vi "test Get All Parameters.vi"(8 "error in":errorcluster, 11 "TestCase in":refnum<class "Scripting.lvclass">) -> (0 "error out":errorcluster, 3 "TestCase out":refnum<class "Scripting.lvclass">)   [LabVIEW 2020, in "Scripting.lvclass"]
uses:
  Scripting.lvclass
  <vilib>/addons/_JKI Toolkits/VI Tester/TestCase.llb/TestCase.lvclass
  Scripting/AIM/AIM ARINC 429 Scripting.lvlib
  Shared/Transfer Type.ctl
  <vilib>/NI/NI VeriStand Encoding and Decoding/Encoding.ctl
  <vilib>/NI/NI VeriStand Encoding and Decoding/Encoding and Decoding.lvlib
  Shared/Parameter Definition.ctl
  Shared/VS Channel Definition for Parameter.ctl
  Shared/VS Channels Definition for Label.ctl
  Shared/Direction.ctl
  Shared/Transfer Speed.ctl
  C:/Program Files (x86)/National Instruments/LabVIEW 2020/vi.lib/addons/_JKI Toolkits/VI Tester/TestCase.llb/TestCase.lvclass
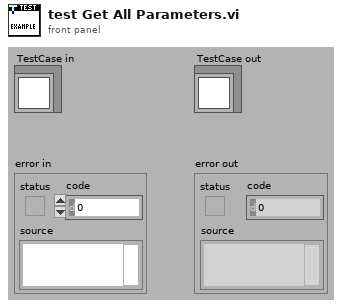
[diagram p1: front panel]
types:
  T1 = typedef "VS Channels Definition for Label.ctl" = cluster{"label (Dec)":u32, "parameters":T2[], "SDI value":u8, "SDI enabled":bool, "transfer type":T5, "create timestamp":bool, "transmit period":u32}
  T2 = typedef "VS Channel Definition for Parameter.ctl" = cluster{"name":string, "unit":string, "Parameter":T3}
  T3 = typedef "Parameter Definition.ctl" = cluster{"start index":i32, "size":i32, "encoding":T4, "signed":bool, "scale multiplier":dbl, "scale offset":dbl, "default value":dbl}
  T4 = typedef "Encoding and Decoding.lvlib/Encoding.ctl" = enum16{"BNR", "BCD", "Discrete"}
  T5 = typedef "Transfer Type.ctl" = enum16{"Scheduled", "Acyclic", "Block", "Strobe"}
  T6 = typedef "Transfer Speed.ctl" = enum16{"LO (12.5 kb/s)", "HI (100 kb/s)"}
  T7 = typedef "Direction.ctl" = enum16{"Rx", "Tx"}
  T8 = typedef "Custom Device API.lvlib/Custom Device Item Ref.ctl" = u64
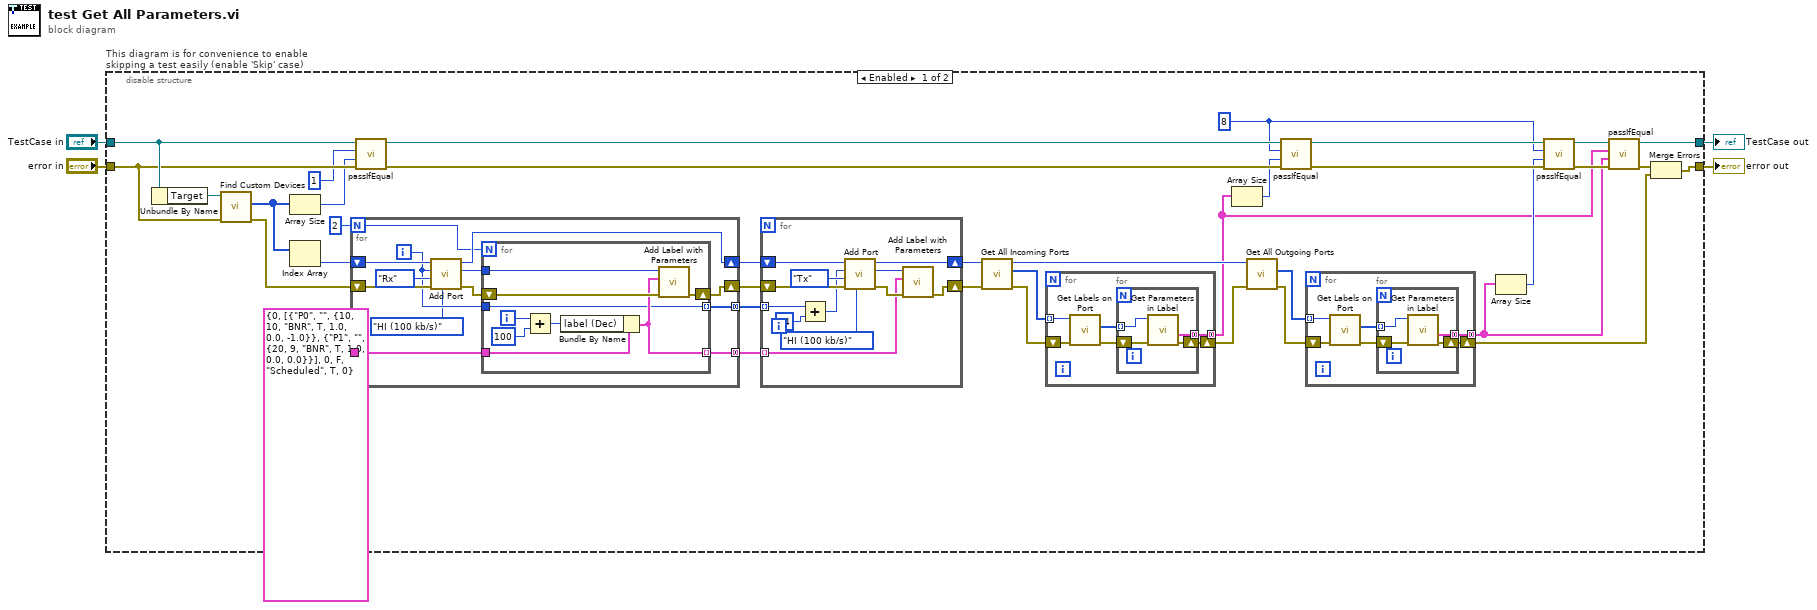
[diagram p0: block diagram]
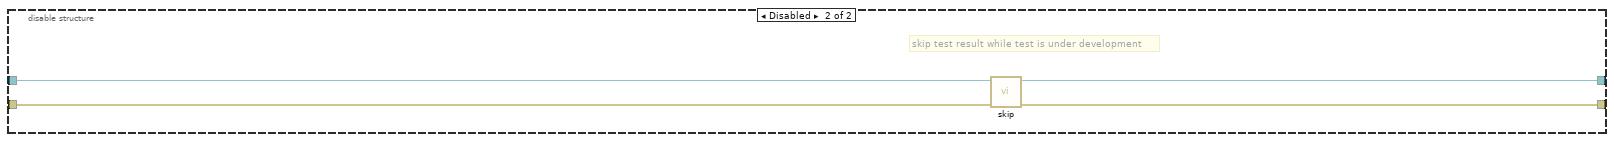
[diagram p2: hidden frame]
diagram:
  n1 = disable-structure "This diagram is for convenience to enable skipping a test easily (enable 'Skip' case)" shown="Enabled" {
    disable-tunnel: "TestCase in" -> [w40 w99]
    disable-tunnel: [w32 w97] -> w1
    disable-tunnel: [w33 w98] -> w3
    disable-tunnel: "error in" -> [w39 w96]
    frame Enabled {
      w7 = 8 ("size(s)")
      n2 = Unbundle By Name(w40) -> ("Target"=w41:refnum<k24>)
      n3 = call "Find Custom Devices.vi"("error in"=w39, "target in"=w41) -> ("error out"=w15:errorcluster, "AIM ARINC 429 custom devices"=w18:u64[])  [unwired: 7 in, 1 out]
      n4 = Array Size(array=w18) -> (size(s)=w37:i32)
      n5 = Index Array(array=w18) -> (element=w17:u64)  [unwired: 1 in]
      n6 = for {
        N: 2 -> [w55]
        shift-right: [w60] -> w11
        shift-left: w17 -> [w64]
        shift-right: [w61] -> w10
        shift-left: w15 -> [w62]
        tunnel: T1 {"label (Dec)"=0, "parameters"=[{"name"="P0", "unit"="", "Parameter"={"start index"=10, "size"=10, "encoding"=enum."BNR", "signed"=TRUE, "scale multiplier"=1.0, "scale offset"=0.0, "default value"=-1.0}}, {"name"="P1", "unit"="", "Parameter"={"start index"=20, "size"=9, "encoding"=enum."BNR", "signed"=TRUE, "scale multiplier"=1.0, "scale offset"=0.0, "default value"=0.0}}], "SDI value"=0, "SDI enabled"=FALSE, "transfer type"=enum."Scheduled", "create timestamp"=TRUE, "transmit period"=0} ("label") -> [w59]
        tunnel: [w58] -> w9 mode=concatenating
        tunnel: [w56] -> w8 mode=concatenating
        i -> [w57]
        n7 = call "Add Port.vi"("speed"=Transfer_Speed."HI (100 kb/s)", "error in"=w62, "direction"=Direction."Rx", "port number"=w57, "AIM ARINC 429 custom device in"=w64) -> ("error out"=w65:errorcluster, "port"=w66:T8, "AIM ARINC 429 custom device out"=w60:T8)  [unwired: 4 in]
        n8 = for {
          N: w55 -> [_]
          tunnel: w66 -> [w75]
          shift-right: [w73] -> w61
          shift-left: w65 -> [w74]
          tunnel: w59 -> [w72]
          tunnel: [w71] -> w58 mode=indexing
          tunnel: w57 -> [w67]
          tunnel: [w67] -> w56 mode=indexing
          i -> [w70]
          n9 = Add(x=w70, y=100) -> (x+y=w69:i32)
          n10 = Bundle By Name(cluster=w72, "label (Dec)"=w69) -> (w71:T1)
          n11 = call "Add Label with Parameters.vi"("error in"=w74, "label"=w71, "port ref"=w75) -> ("error out"=w73:errorcluster)  [unwired: 7 in, 1 out]
        }
      }
      n12 = call-dynamic "passIfEqual.vi"("error in (no error)"=w39, "y"=w37, "x"=1 ("size(s)"), "TestCase in"=w40) -> ("error out"=w35:errorcluster, "TestCase out"=w36:refnum<class "Scripting.lvclass">)  [unwired: 6 in]
      n13 = for {
        shift-right: [w50] -> w13
        shift-left: w11 -> [w51]
        shift-right: [w47] -> w12
        shift-left: w10 -> [w48]
        tunnel: w9 -> [w44] mode=indexing
        tunnel: w8 -> [w43] mode=indexing
        n14 = Add(x=w43, y=24 ("x")) -> (x+y=w45:i32)
        n15 = call "Add Port.vi"("speed"=Transfer_Speed."HI (100 kb/s)", "error in"=w48, "direction"=Direction."Tx", "port number"=w45, "AIM ARINC 429 custom device in"=w51) -> ("error out"=w52:errorcluster, "port"=w53:T8, "AIM ARINC 429 custom device out"=w50:T8)  [unwired: 4 in]
        n16 = call "Add Label with Parameters.vi"("error in"=w52, "label"=w44, "port ref"=w53) -> ("error out"=w47:errorcluster)  [unwired: 7 in, 1 out]
      }
      n17 = call "Get All Incoming Ports.vi"("error in"=w12, "AIM ARINC 429 custom device in"=w13) -> ("error out"=w27:errorcluster, "incoming ports"=w26:T8[], "AIM ARINC 429 custom device out"=w34:T8)  [unwired: 7 in]
      n18 = for {
        tunnel: [w90] -> w5 mode=concatenating
        shift-right: [w91] -> w30
        shift-left: w27 -> [w89]
        tunnel: w26 -> [w86] mode=indexing
        n19 = call "Get Labels on Port.vi"("error in"=w89, "port in"=w86) -> ("error out"=w88:errorcluster, "labels"=w87:T8[])  [unwired: 6 in, 2 out]
        n20 = for {
          tunnel: [w94] -> w90 mode=concatenating
          shift-right: [w95] -> w91
          shift-left: w88 -> [w93]
          tunnel: w87 -> [w92] mode=indexing
          n21 = call "Get Parameters in Label.vi"("error in"=w93, "label in"=w92) -> ("error out"=w95:errorcluster, "parameter definitions"=w94:T3[])  [unwired: 6 in, 2 out]
        }
      }
      n22 = Array Size(array=w5) -> (size(s)=w20:i32)
      n23 = call "Get All Outgoing Ports.vi"("error in"=w30, "AIM ARINC 429 custom device in"=w34) -> ("error out"=w22:errorcluster, "outgoing ports"=w23:T8[])  [unwired: 7 in, 1 out]
      n24 = call-dynamic "passIfEqual.vi"("error in (no error)"=w35, "y"=w20, "x"=w7, "TestCase in"=w36) -> ("error out"=w28:errorcluster, "TestCase out"=w29:refnum<class "Scripting.lvclass">)  [unwired: 6 in]
      n25 = for {
        tunnel: [w80] -> w6 mode=concatenating
        shift-right: [w81] -> w21
        shift-left: w22 -> [w79]
        tunnel: w23 -> [w76] mode=indexing
        n26 = call "Get Labels on Port.vi"("error in"=w79, "port in"=w76) -> ("error out"=w78:errorcluster, "labels"=w77:T8[])  [unwired: 6 in, 2 out]
        n27 = for {
          tunnel: [w84] -> w80 mode=concatenating
          shift-right: [w85] -> w81
          shift-left: w78 -> [w83]
          tunnel: w77 -> [w82] mode=indexing
          n28 = call "Get Parameters in Label.vi"("error in"=w83, "label in"=w82) -> ("error out"=w85:errorcluster, "parameter definitions"=w84:T3[])  [unwired: 6 in, 2 out]
        }
      }
      n29 = Array Size(array=w6) -> (size(s)=w19:i32)
      n30 = call-dynamic "passIfEqual.vi"("error in (no error)"=w28, "y"=w19, "x"=w7, "TestCase in"=w29) -> ("error out"=w24:errorcluster, "TestCase out"=w25:refnum<class "Scripting.lvclass">)  [unwired: 6 in]
      n31 = call-dynamic "passIfEqual.vi"("error in (no error)"=w24, "y"=w6, "x"=w5, "TestCase in"=w25) -> ("error out"=w31:errorcluster, "TestCase out"=w32:refnum<class "Scripting.lvclass">)  [unwired: 6 in]
      n32 = Merge Errors(w31, w21) -> (w33:errorcluster)
    }
    frame Disabled {
      # "skip test result while test is under development"
      n33 = call <vilib>:"skip.vi"("error in (no error)"=w96, "TestCase in"=w99) -> ("error out"=w98:errorcluster, "TestCase out"=w97:refnum<class "Scripting.lvclass">)  [unwired: 8 in]
    }
  }
  "error out" <- w3
  "TestCase out" <- w1
